vi "Run Tests in UI.vi"(8 "error in (no error)":errorcluster, 10 "Path":path, 11 "Application":refnum<vi>) -> (0 "error out":errorcluster)   [LabVIEW 2020, in "Project Provider.lvlib"]
uses:
  Project Provider.lvlib
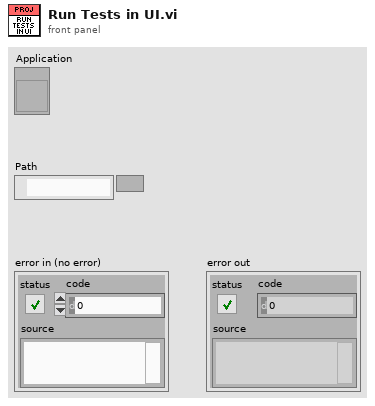
[diagram p1: front panel]
types:
  T1 = enum32{"Invalid", "Standard", "Closed", "Hidden", "Minimized", "Maximized"}
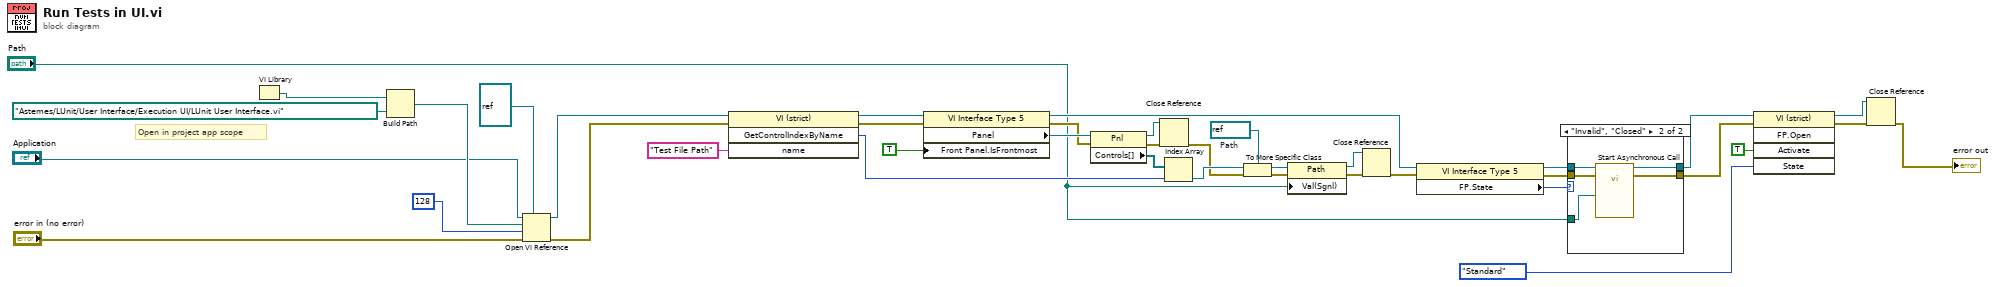
[diagram p0: block diagram]
diagram:
  w23 = refnum<vi> refnum  # Path
  # "Open in project app scope"
  n1 = VI Library() -> (path=w31:path)
  n2 = Build Path(base path=w31, name or relative path=path "Astemes/LUnit/User Interface/Execution UI/LUnit User Interface.vi" ("Relative Path from 1 to 2")) -> (appended path=w36:path)
  n3 = Open VI Reference(type specifier VI Refnum (for type only)=refnum<vi> refnum, application reference (local)="Application", vi path=w36, options=128, error in (no error)="error in (no error)") -> (vi reference=w11:refnum<vi>, error out=w10:errorcluster)  [unwired: 1 in]
  n4 = invoke class="VI (strict)" method="GetControlIndexByName"(reference=w11, error in=w10, "name"="Test File Path" ("Control Name")) -> (reference out=w27:refnum<vi>, error out=w17:errorcluster, "GetControlIndexByName"=w24:i32)  [unwired: 1 in, 1 out]
  n5 = property class="VI Interface Type 5"(reference=w27, error in=w17, "Front Panel.IsFrontmost"=TRUE ("Front Panel Window:Is Frontmost")) -> (reference out=w4:refnum<vi>, error out=w18:errorcluster, "Panel"=w28:refnum<vi>)
  n6 = property class="Pnl"(reference=w28, error in=w18) -> (reference out=w14:refnum<vi>, error out=w19:errorcluster, "Controls[]"=w25:refnum<vi>[])
  n7 = Close Reference(reference=w14, error in (no error)=w19) -> (error out=w15:errorcluster)
  n8 = Index Array(array=w25, index=w24) -> (element=w21:refnum<vi>)
  n9 = To More Specific Class(target class=w23, reference=w21, error in=w15) -> (specific class reference=w22:refnum<vi>, error out=w20:errorcluster)
  n10 = property class="Path"(reference=w22, error in=w20, "Val(Sgnl)"="Path") -> (reference out=w13:refnum<vi>, error out=w16:errorcluster)
  n11 = Close Reference(reference=w13, error in (no error)=w16) -> (error out=w6:errorcluster)
  n12 = property class="VI Interface Type 5"(reference=w4, error in=w6) -> (reference out=w8:refnum<vi>, error out=w9:errorcluster, "FP.State"=w7:T1)
  n13 = case shown="\"Invalid\", \"Closed\"" w7 {
    tunnel: w9 -> [w41 w46]
    tunnel: w8 -> [w40 w45]
    tunnel: [w41 w43] -> w5
    tunnel: [w40 w44] -> w3
    tunnel: "Path" -> [_ w42]
    frame Default {
    }
    frame "Invalid", "Closed" {
      n14 = call-by-ref "Start Asynchronous Call"(reference=w45, error in=w46, "Test File Path"=w42) -> (reference out=w44:refnum<vi>, error out=w43:errorcluster)  [unwired: 11 in]
    }
  }
  n15 = invoke class="VI (strict)" method="FP.Open"(reference=w3, error in=w5, "Activate"=TRUE ("Activate?"), "State"=T1."Standard") -> (reference out=w35:refnum<vi>, error out=w34:errorcluster)  [unwired: 1 in, 3 out]
  n16 = Close Reference(reference=w35, error in (no error)=w34) -> (error out=→"error out":errorcluster)
